vi "Scripting_UpdateViFromTemplate.vi"(0 "ViRef":refnum<vi>, 1 "TemplateVI(Path or Ref)":variant, 5 "error in (no error)":errorcluster) -> (15 "TemplateVersionUsed":string, 19 "error out":errorcluster={"status"=TRUE, "code"=1055, "source"="Property Node in Scripting_ConvertBaseClassToSubClass.vi"})   [LabVIEW 2020]
uses:
  <vilib>/Utility/miscctls.llb/LVRectTypeDef.ctl
  <vilib>/Utility/miscctls.llb/LVPositionTypeDef.ctl
  <vilib>/Utility/traverseref.llb/TRef TravTarget.ctl
  b5d46679-8400-4ee0-8a03-e36cc4015ed4.vi
  Scripting.lvclass
  <vilib>/Utility/traverseref.llb/VI Scripting - Traverse.lvlib
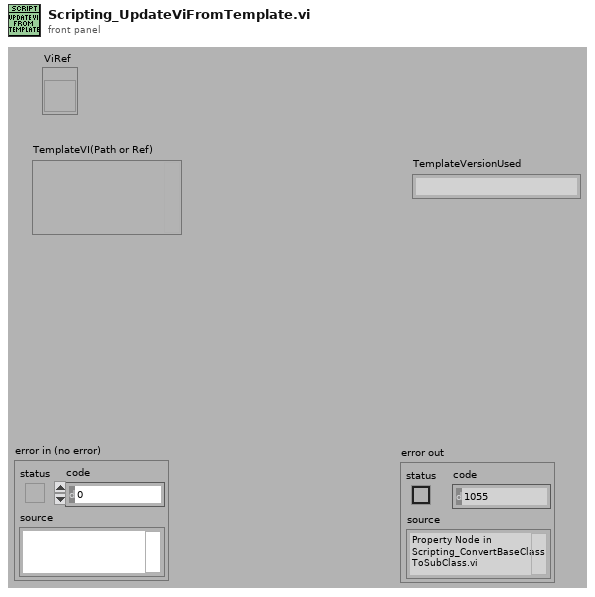
[diagram p1: front panel]
types:
  T1 = typedef "LVRectTypeDef.ctl" = cluster{"Left":i16, "Top":i16, "Right":i16, "Bottom":i16}
  T2 = typedef "LVPositionTypeDef.ctl" = cluster{"Left":i32, "Top":i32}
  T3 = cluster{"ViRef":refnum<vi>, "TemplateRef":refnum<vi>, "ConnectorPaneSettings":cluster{i32, "Wire Rule":enum16{"Invalid Wire Rule", "Required", "Recommended", "Optional", "Dynamic Dispatch"}}[], "ConnectorPaneControlsLabels":string[], "ViClassPath":path, "TemplateViClassPath":path, "ViRootBaseClassPath":path, "TemplateRootBaseClassPath":path, "ClassName":string, "TemplateMemberDataPath":path, "TemplateFile":path, "TemplateVersionUsed":string, "Class":refnum<vi>, "TemplateClassName":string, "permissions":i16, "TemplateClass":refnum<vi>, "Master Bounds Rect":T1, "Visible":bool[], "Controls":refnum<vi>[], "Positions":T2[], "CtrlsNotOnCP":string[]}
  T4 = enum32{"invalid lock state", "Not Locked", "Locked (No Password)", "Password-protected"}
  T5 = typedef "TRef TravTarget.ctl" = enum16{"FP", "BD", "Other"}
  T6 = enum32{"invalid VI type", "Standard VI", "Control VI", "Global VI", "Polymorphic VI", "Configuration VI", "SubSystem", "Facade VI", "Method VI", "Statechart Diagram VI"}
  T7 = enum32{"invalid VI type", "Standard VI", "Control VI", "Global VI", "Polymorphic VI", "Configuration VI", "SubSystem", "Facade VI", "Method VI"}
  T8 = cluster{"Major":u16, "Minor":u16, "Fix":u16, "Build":u16}
  T9 = enum16{"Invalid Wire Rule", "Required", "Recommended", "Optional", "Dynamic Dispatch"}[]
  T10 = cluster{i32, "Wire Rule":enum16{"Invalid Wire Rule", "Required", "Recommended", "Optional", "Dynamic Dispatch"}}
  T11 = cluster{"Position":T2, "Label.Text":string, "Visible":bool, cluster{i32, "Wire Rule":enum16{"Invalid Wire Rule", "Required", "Recommended", "Optional", "Dynamic Dispatch"}}}
  T12 = cluster{"Position":T2, "Label.Text":string, "Visible":bool, cluster{i32, "Wire Rule":enum16{"Invalid Wire Rule", "Required", "Recommended", "Optional", "Dynamic Dispatch"}}}[]
  T13 = cluster{i32, "Wire Rule":enum16{"Invalid Wire Rule", "Required", "Recommended", "Optional", "Dynamic Dispatch"}}[]
  T14 = cluster{"Position":T2, refnum<vi>, "Label.Text":string}
  T15 = cluster{"Position":T2, refnum<vi>, "Label.Text":string}[]
  T16 = enum16{"Invalid Wire Rule", "Required", "Recommended", "Optional", "Dynamic Dispatch"}
  T17 = enum32{"Bad", "Idle", "Run top level", "Running"}
  T18 = typedef "LVPointTypeDef.ctl" = cluster{"Horizontal":i16, "Vertical":i16}
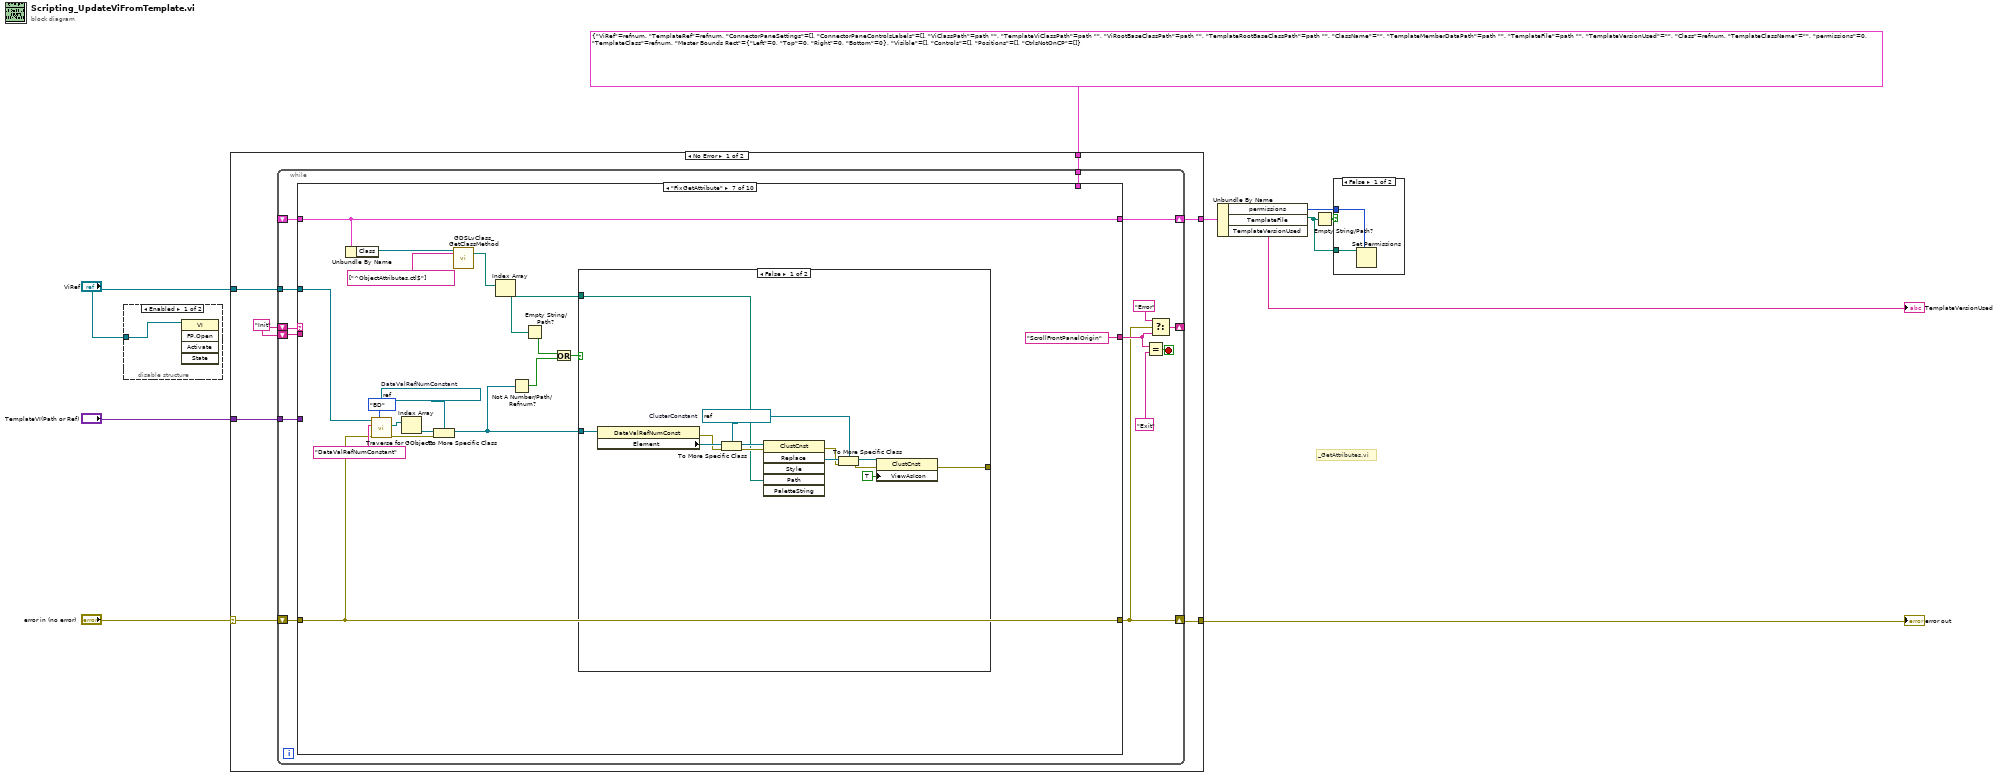
[diagram p0: block diagram]
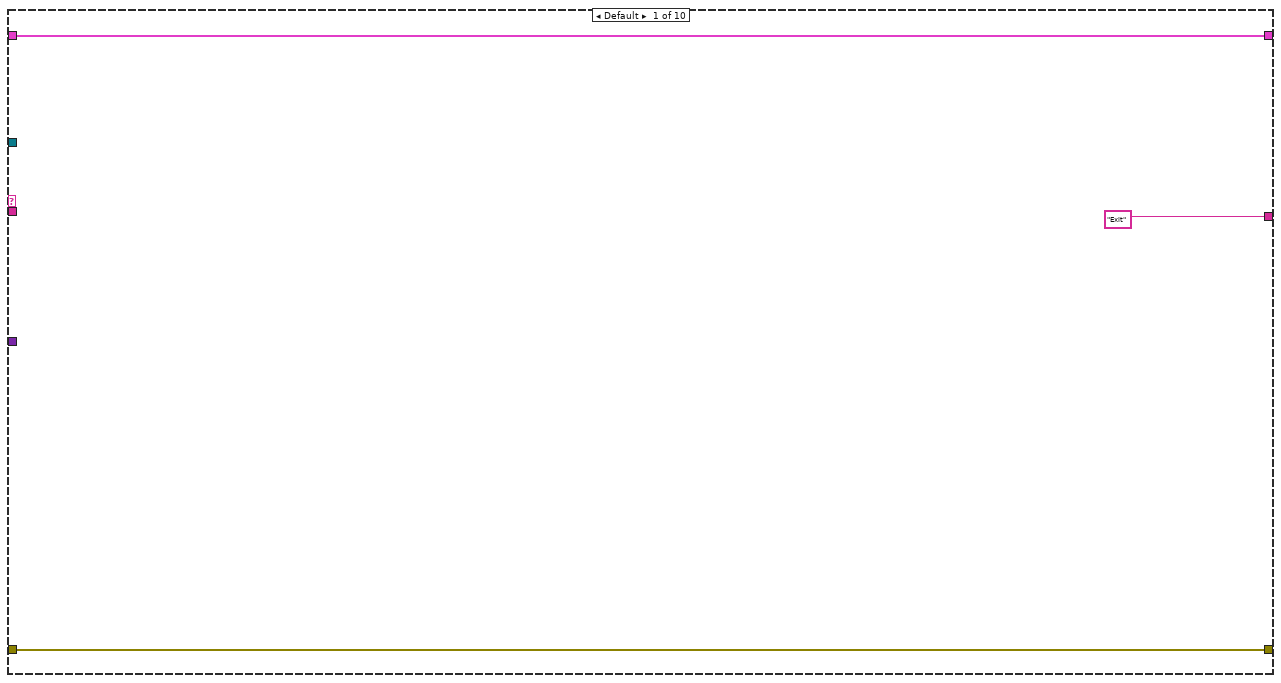
[diagram p4: hidden frame]
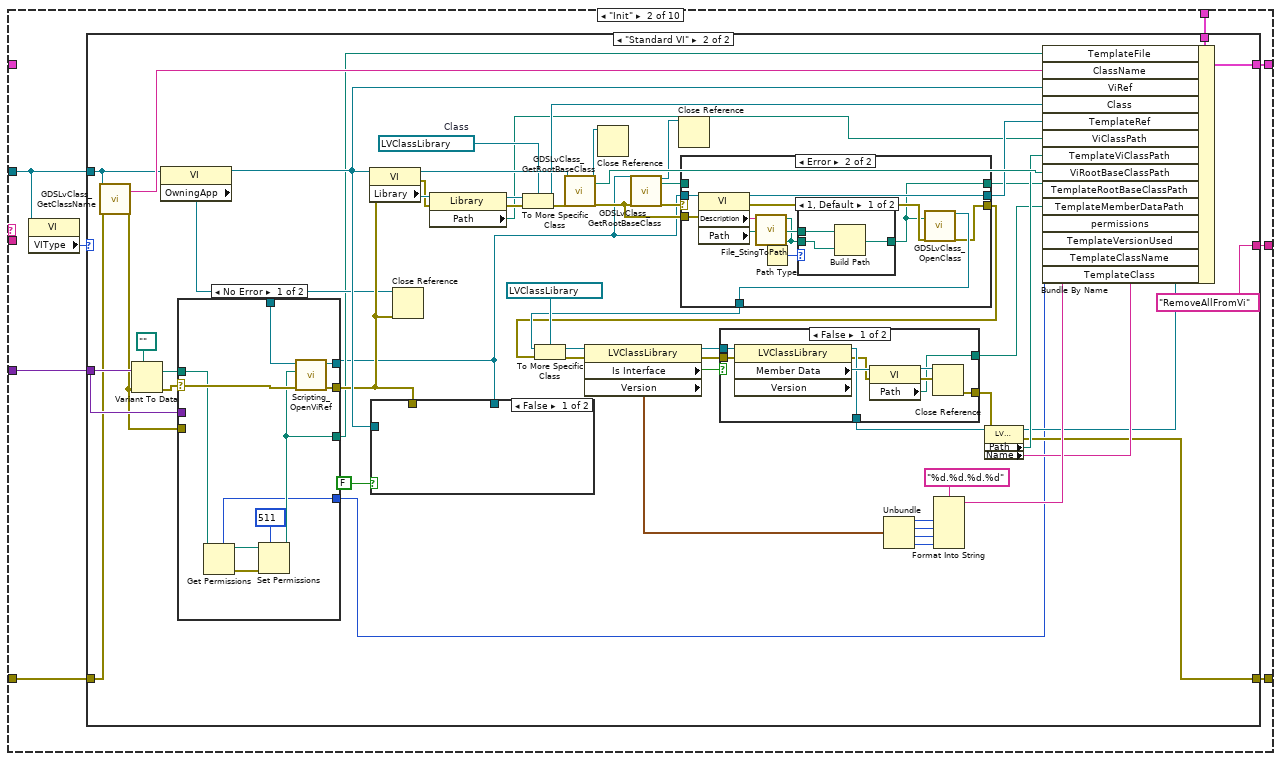
[diagram p5: hidden frame]
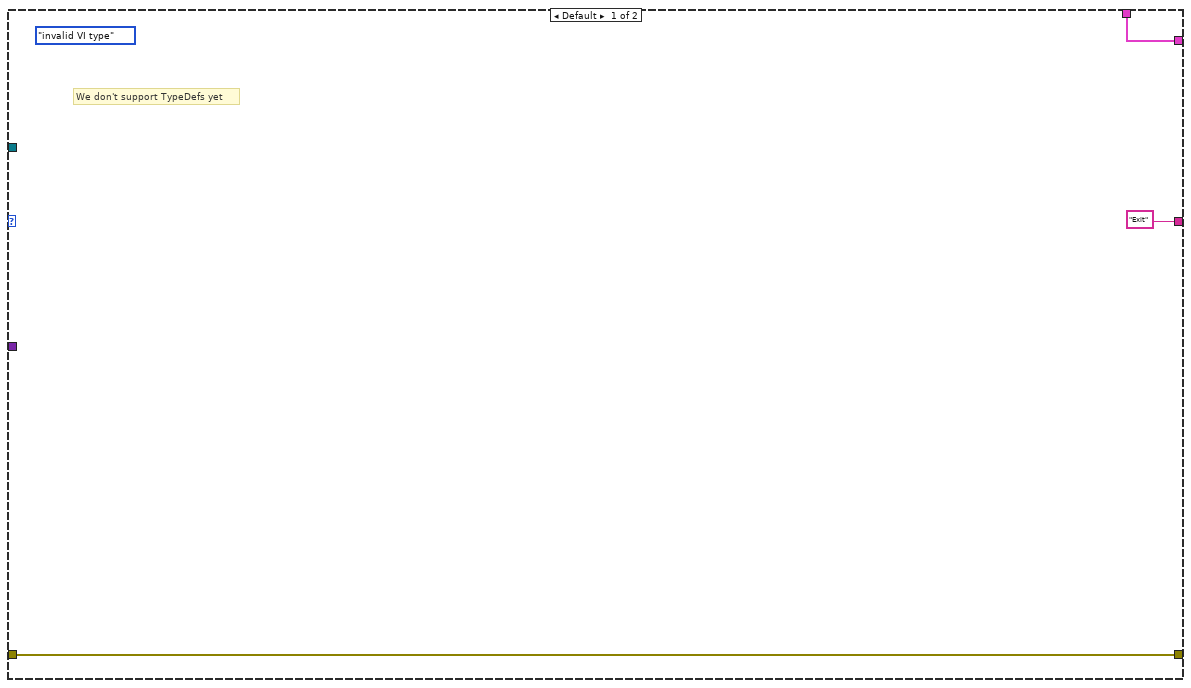
[diagram p6: hidden frame]
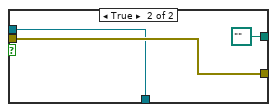
[diagram p7: hidden frame]
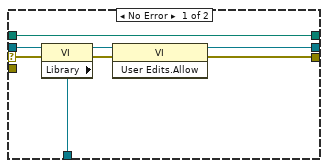
[diagram p8: hidden frame]
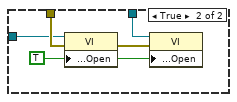
[diagram p10: hidden frame]
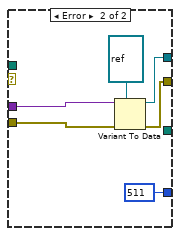
[diagram p11: hidden frame]
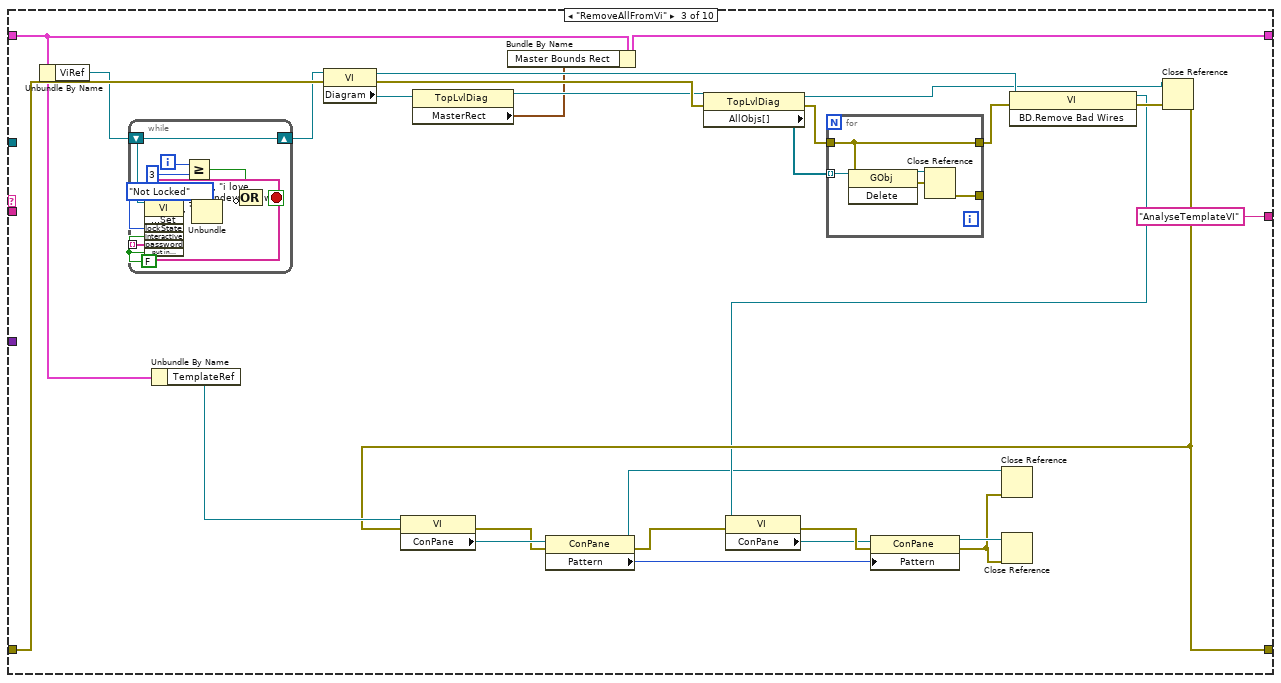
[diagram p12: hidden frame]
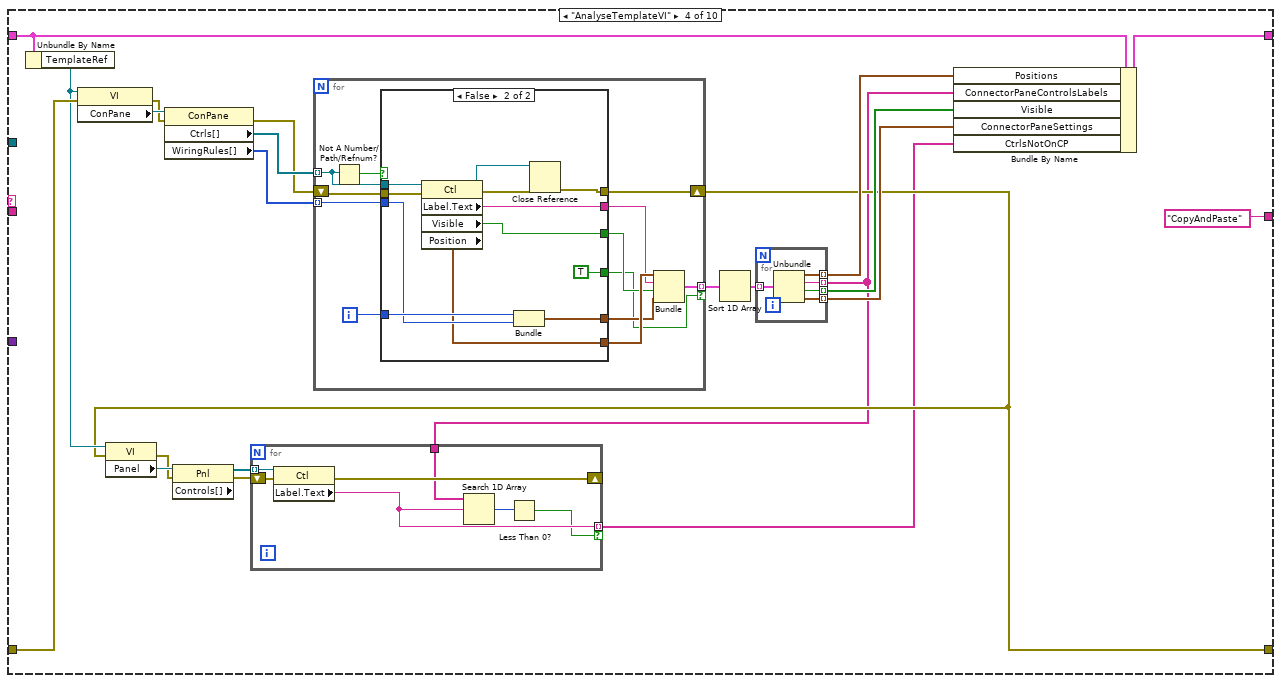
[diagram p13: hidden frame]
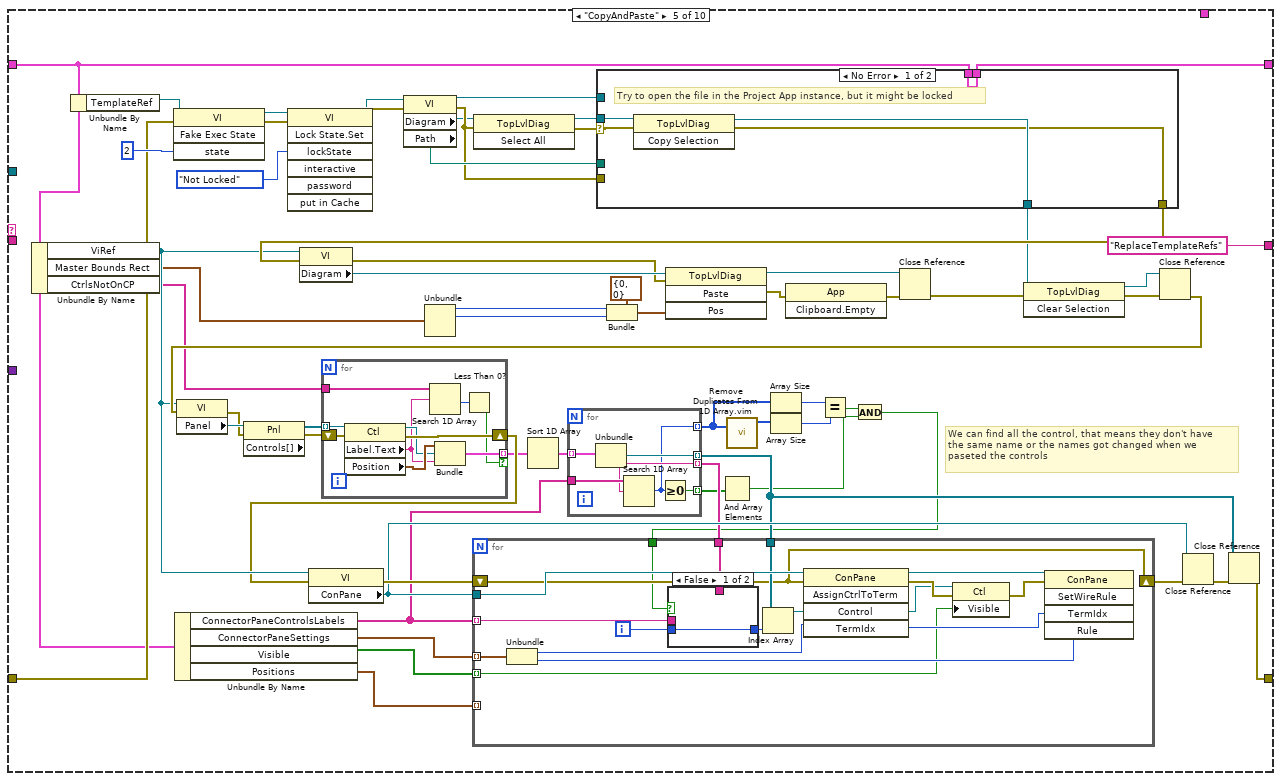
[diagram p15: hidden frame]
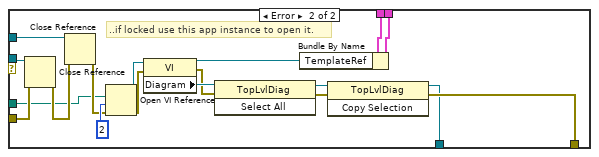
[diagram p16: hidden frame]
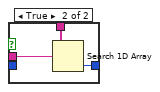
[diagram p17: hidden frame]
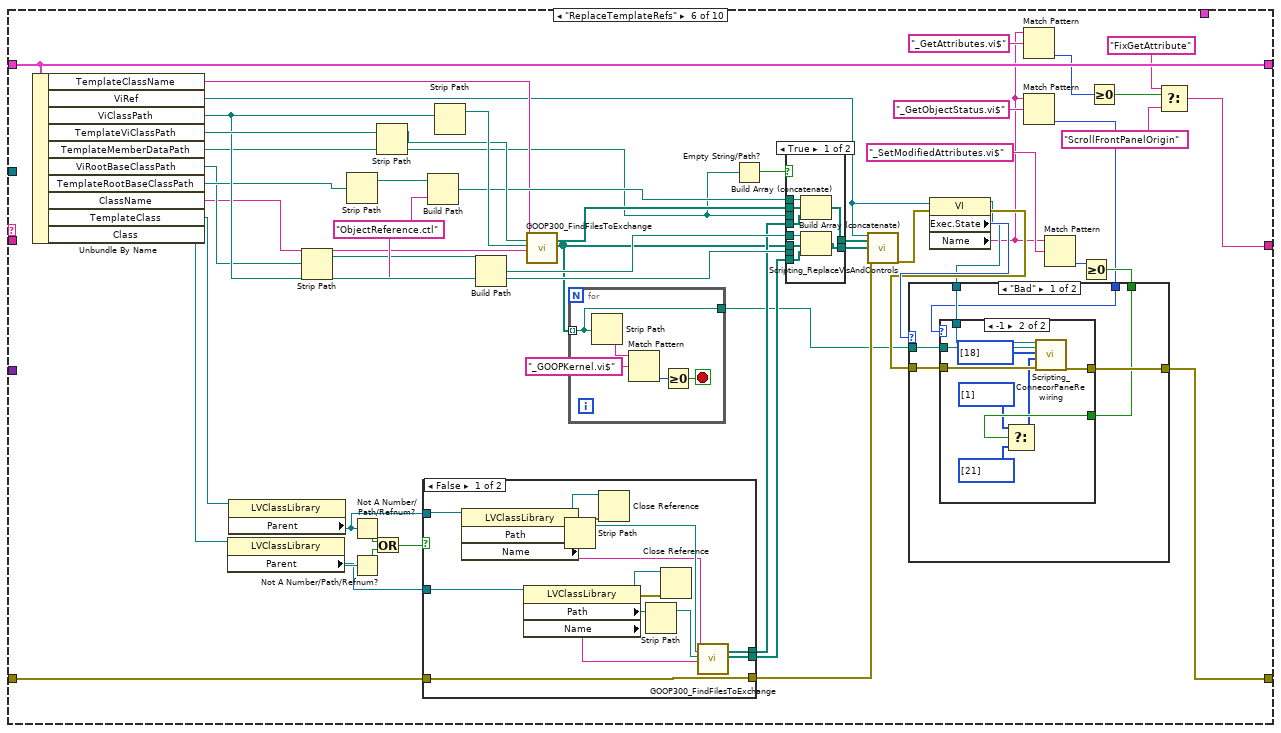
[diagram p18: hidden frame]
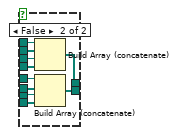
[diagram p19: hidden frame]
diagram:
  # "_GetAttributes.vi"
  n1 = disable-structure shown="Enabled" {
    disable-tunnel: "ViRef" -> [w11 _]
    frame Enabled {
      n2 = invoke class="VI" method="FP.Open"(reference=w11) -> ()  [unwired: 4 in, 5 out]
    }
    frame Disabled {
    }
  }
  n3 = case shown="No Error" "error in (no error)" {
    selector: "error in (no error)" -> [w13 w635]
    tunnel: [w18 w635] -> w10
    tunnel: T3 {"ViRef"=refnum, "TemplateRef"=refnum, "ConnectorPaneSettings"=[], "ConnectorPaneControlsLabels"=[], "ViClassPath"=path "", "TemplateViClassPath"=path "", "ViRootBaseClassPath"=path "", "TemplateRootBaseClassPath"=path "", "ClassName"="", "TemplateMemberDataPath"=path "", "TemplateFile"=path "", "TemplateVersionUsed"="", "Class"=refnum, "TemplateClassName"="", "permissions"=0, "TemplateClass"=refnum, "Master Bounds Rect"={"Left"=0, "Top"=0, "Right"=0, "Bottom"=0}, "Visible"=[], "Controls"=[], "Positions"=[], "CtrlsNotOnCP"=[]} -> [w17 _]
    tunnel: "ViRef" -> [w16 _]
    tunnel: "TemplateVI(Path or Ref)" -> [w15 _]
    tunnel: [w12 _] -> w6
    frame No Error {
      w14 = "Init"
      n4 = while {
        shift-right: [w20] -> w18
        shift-left: w13 -> [w22]
        shift-right: [w32] -> _
        shift-left: w14 -> [w27]
        shift-right: [w21] -> w12
        shift-left: _ -> [w26]
        tunnel: w16 -> [w24]
        tunnel: w17 -> [w25]
        tunnel: w15 -> [w23]
        shift-left: w14 -> [w19]
        stop <- w31 stop-if-true
        n5 = case shown="\"FixGetAttribute\"" w27 {
          tunnel: w22 -> [w35 w39 w186 w221 w310 w394 w500 w559 w590 w596]
          tunnel: [w35 w38 w167 w205 w280 w392 w500 w559 w589 w599] -> w20
          tunnel: ["Exit" w43 "AnalyseTemplateVI" "CopyAndPaste" "ReplaceTemplateRefs" w381 "ScrollFrontPanelOrigin" "SaveVI" "CloseReferences" "Exit"] -> w28
          tunnel: [w33 w42 w173 w222 w302 w393 w498 w528 w592 w595] -> w21
          tunnel: w26 -> [w33 _ w171 w223 w296 w393 w498 w528 w592 w595]
          tunnel: w24 -> [_ w37 _ _ _ _ w501 w521 _ w604]
          tunnel: w25 -> [_ w41 _ _ _ _ _ _ _ _]
          tunnel: w23 -> [_ w40 _ _ _ _ _ _ _ w606]
          tunnel: w19 -> [_ _ _ _ _ _ _ _ _ w594]
          frame Default {
          }
          frame "Init" {
            n6 = property class="VI"(reference=w37) -> ("VIType"=w36:T6)  [unwired: 1 in, 2 out]
            n7 = case shown="\"Standard VI\"" w36 {
              tunnel: ["Exit" "RemoveAllFromVi"] -> w43
              tunnel: [w46 w102] -> w42
              tunnel: w41 -> [w46 w101]
              tunnel: w40 -> [_ w97]
              tunnel: w39 -> [w44 w88]
              tunnel: [w44 w64] -> w38
              tunnel: w37 -> [_ w62]
              frame Default {
                (unwired) T7."invalid VI type" ("VIType")
                # "We don't support TypeDefs yet"
              }
              frame "Standard VI" {
                w68 = refnum<vi> refnum  # Class
                n8 = call "GDSLvClass_GetClassName.vi"("ViRef/Path,LvClassRef/Path"=w62, "error in (no error)"=w88) -> ("ClassName(without .lvclass)"=w87:string, "error out"=w85:errorcluster)  [unwired: 15 in, 1 out]
                n9 = Variant To Data(error in=w85, type=path "", Variant=w97) -> (data=w98:path, error out=w99:errorcluster)
                n10 = property class="VI"(reference=w62) -> (reference out=w82:refnum<vi>, "OwningApp"=w80:refnum<vi>)  [unwired: 1 in, 1 out]
                n11 = case shown="No Error" w99 {
                  selector: w99 -> [w152 _]
                  tunnel: w98 -> [w145 _]
                  tunnel: [w151 w155] -> w53
                  tunnel: [w150 w154] -> w81
                  tunnel: w85 -> [_ w158]
                  tunnel: w97 -> [_ w157]
                  tunnel: w80 -> [w149 _]
                  tunnel: [w147 _] -> w77
                  tunnel: [w143 i16 511 ("permissions")] -> w60
                  frame No Error {
                    n12 = Get Permissions(11:w145) -> (0:w146:errorcluster, 3:w144:path, 5:w143:i16)  [unwired: 1 in, 2 out]
                    n13 = Set Permissions(7:i16 511 ("permissions"), 8:w146, 11:w144) -> (3:w147:path)  [unwired: 2 in, 1 out]
                    n14 = call "Scripting_OpenViRef.vi"("error in"=w152, "ViPath/ViName/Viref"=w147, "AppRef"=w149) -> ("error out"=w150:errorcluster, "vi reference"=w151:refnum<vi>)  [unwired: 6 in, 1 out]
                  }
                  frame Error {
                    n15 = Variant To Data(error in=w158, type=refnum<vi> refnum ("ViRef"), Variant=w157) -> (data=w155:refnum<vi>, error out=w154:errorcluster)
                  }
                }
                n16 = property class="VI"(reference=w82, error in=w81) -> (reference out=w95:refnum<vi>, error out=w84:errorcluster, "Library"=w96:refnum<vi>)
                n17 = case shown="False" FALSE {
                  tunnel: w81 -> [_ w140]
                  tunnel: w53 -> [_ w139]
                  tunnel: w82 -> [_ w138]
                  frame False {
                  }
                  frame True {
                    w141 = TRUE ("Front Panel Window:Open")
                    n18 = property class="VI"(reference=w138, error in=w140, "Front Panel.Open"=w141) -> (error out=w142:errorcluster)  [unwired: 1 out]
                    n19 = property class="VI"(reference=w139, error in=w142, "Front Panel.Open"=w141) -> ()  [unwired: 2 out]
                  }
                }
                n20 = Close Reference(reference=w80, error in (no error)=w81) -> ()  [unwired: 1 out]
                n21 = property class="Library"(reference=w96, error in=w84) -> (reference out=w70:refnum<vi>, error out=w69:errorcluster, "Path"=w59:path)
                n22 = To More Specific Class(target class=w68, reference=w70, error in=w69) -> (specific class reference=w66:refnum<vi>, error out=w67:errorcluster)
                n23 = call "GDSLvClass_GetRootBaseClass.vi"("ViRef/Path,LvClassRef/Path"=w95, "error in (no error)"=w67) -> ("RootBaseClassRef"=w94:refnum<vi>, "RootBaseClassPath"=w93:path, "error out"=w57:errorcluster)  [unwired: 11 in, 4 out]
                n24 = Close Reference(reference=w94) -> ()  [unwired: 1 in, 1 out]
                n25 = call "GDSLvClass_GetRootBaseClass.vi"("ViRef/Path,LvClassRef/Path"=w53, "error in (no error)"=w57) -> ("RootBaseClassRef"=w61:refnum<vi>, "RootBaseClassPath"=w56:path, "error out"=w58:errorcluster)  [unwired: 11 in, 4 out]
                n26 = Close Reference(reference=w61) -> ()  [unwired: 1 in, 1 out]
                n27 = case shown="Error" w58 {
                  selector: w58 -> [w117 _]
                  tunnel: [w123 w129] -> w91
                  tunnel: [w122 w133] -> w79
                  tunnel: [w120 w128] -> w78
                  tunnel: w53 -> [w118 w133]
                  tunnel: w57 -> [_ w132]
                  tunnel: w56 -> [w116 _]
                  tunnel: [w116 w124] -> w55
                  frame No Error {
                    n28 = property class="VI"(reference=w118, error in=w117) -> (reference out=w119:refnum<vi>, error out=w121:errorcluster, "Library"=w123:refnum<vi>)
                    n29 = invoke class="VI" method="User Edits.Allow"(reference=w119, error in=w121) -> (reference out=w122:refnum<vi>, error out=w120:errorcluster)  [unwired: 1 in, 1 out]
                  }
                  frame Error {
                    n30 = property class="VI"(reference=w133, error in=w132) -> (error out=w130:errorcluster, "Description"=w131:string, "Path"=w127:path)  [unwired: 1 out]
                    n31 = call "File_StingToPath.vi"("Description"=w131) -> ("Path"=w126:path)  [unwired: 10 in]
                    n32 = Path Type(1:w126) -> (0:w125:i16)
                    n33 = case shown="1, Default" w125 {
                      tunnel: w126 -> [w134 w137]
                      tunnel: [w136 w137] -> w124
                      tunnel: w127 -> [w135 _]
                      frame 1, Default {
                        n34 = Build Path(base path=w135, name or relative path=w134) -> (appended path=w136:path)
                      }
                      frame 0 {
                      }
                    }
                    n35 = call "GDSLvClass_OpenClass.vi"("ClassToOpen"=w124, "error in (no error)"=w130) -> ("LVClass.Open"=w129:refnum<vi>, "error out"=w128:errorcluster)  [unwired: 16 in]
                  }
                }
                n36 = To More Specific Class(target class=refnum<vi> refnum ("LVClass.Open"), reference=w91, error in=w78) -> (specific class reference=w52:refnum<vi>, error out=w51:errorcluster)
                n37 = property class="LVClassLibrary"(reference=w52, error in=w51) -> (reference out=w50:refnum<vi>, error out=w49:errorcluster, "Is Interface"=w47:bool, "Version"=w48:T8)
                n38 = case shown="False" w47 {
                  tunnel: [w110 w113] -> w90
                  tunnel: [w109 w115] -> w89
                  tunnel: [w106 path "" ("Path")] -> w54
                  tunnel: w50 -> [w105 w113]
                  tunnel: w49 -> [w104 w115]
                  frame False {
                    n39 = property class="LVClassLibrary" props=["Member Data", "Version"](reference=w105, error in=w104) -> (reference out=w110:refnum<vi>, error out=w108:errorcluster, "Member Data"=w111:refnum<vi>)  [unwired: 1 out]
                    n40 = property class="VI"(reference=w111, error in=w108) -> (reference out=w107:refnum<vi>, error out=w112:errorcluster, "Path"=w106:path)
                    n41 = Close Reference(reference=w107, error in (no error)=w112) -> (error out=w109:errorcluster)
                  }
                  frame True {
                  }
                }
                n42 = Unbundle(w48) -> ("Major"=w76:u16, "Minor"=w75:u16, "Fix"=w74:u16, "Build"=w73:u16)
                n43 = Format Into String(format string="%d.%d.%d.%d", w76, w75, w74, w73) -> (resulting string=w71:string)  [unwired: 2 in, 1 out]
                n44 = property class="LVClassLibrary"(reference=w90, error in=w89) -> (reference out=w63:refnum<vi>, error out=w64:errorcluster, "Path"=w86:path, "Name"=w65:string)
                n45 = Bundle By Name(cluster=w101, "TemplateFile"=w77, "ClassName"=w87, "ViRef"=w82, "Class"=w66, "TemplateRef"=w79, "ViClassPath"=w59, "TemplateViClassPath"=w86, "ViRootBaseClassPath"=w93, "TemplateRootBaseClassPath"=w55, "TemplateMemberDataPath"=w54, "permissions"=w60, "TemplateVersionUsed"=w71, "TemplateClassName"=w65, "TemplateClass"=w63) -> (w102:T3)
              }
            }
          }
          frame "RemoveAllFromVi" {
            n46 = Unbundle By Name(w171) -> ("ViRef"=w177:refnum<vi>)
            n47 = while {
              tunnel: string[] ["goop rules", "i love goteborg", "Endevo Knows Goop!", "kiss"] -> [w195] mode=indexing
              shift-right: [w188] -> w176
              shift-left: w177 -> [w188]
              i -> [w192]
              stop <- w193 stop-if-true
              w196 = FALSE ("Interactive")
              n48 = invoke class="VI" method="Lock State.Set"(reference=w188, "lockState"=T4."Not Locked" ("Lock State"), "interactive"=w196, "password"=w195, "put in Cache"=w196) -> (error out=w194:errorcluster)  [unwired: 2 in, 6 out]
              n49 = Greater Or Equal?(x=w192, y=3) -> (x >= y?=w191:bool)
              n50 = Unbundle(w194) -> ("status"=w189:bool)  [unwired: 2 out]
              n51 = Compound Arithmetic op=OR(w191, invert w189) -> (w193:bool)
            }
            n52 = Unbundle By Name(w171) -> ("TemplateRef"=w168:refnum<vi>)
            n53 = property class="VI"(reference=w176, error in=w186) -> (reference out=w184:refnum<vi>, error out=w181:errorcluster, "Diagram"=w175:refnum<vi>)
            n54 = property class="TopLvlDiag"(reference=w175) -> (reference out=w174:refnum<vi>, "MasterRect"=w172:T1)  [unwired: 1 in, 1 out]
            n55 = Bundle By Name(cluster=w171, "Master Bounds Rect"=w172) -> (w173:T3)
            n56 = property class="TopLvlDiag"(reference=w174, error in=w181) -> (reference out=w179:refnum<vi>, error out=w183:errorcluster, "AllObjs[]"=w182:refnum<vi>[])
            n57 = for {
              tunnel: w183 -> [w200]
              tunnel: w182 -> [w201] mode=indexing
              tunnel: [w200] -> w180
              tunnel: [w198] -> _
              n58 = invoke class="GObj" method="Delete"(reference=w201, error in=w200) -> (reference out=w202:refnum<vi>, error out=w199:errorcluster)  [unwired: 1 in, 1 out]
              n59 = Close Reference(reference=w202, error in (no error)=w199) -> (error out=w198:errorcluster)
            }
            n60 = invoke class="VI" method="BD.Remove Bad Wires"(reference=w184, error in=w180) -> (reference out=w163:refnum<vi>, error out=w185:errorcluster)  [unwired: 1 in, 1 out]
            n61 = Close Reference(reference=w179, error in (no error)=w185) -> (error out=w167:errorcluster)
            n62 = property class="VI"(reference=w168, error in=w167) -> (error out=w169:errorcluster, "ConPane"=w170:refnum<vi>)  [unwired: 1 out]
            n63 = property class="ConPane"(reference=w170, error in=w169) -> (reference out=w161:refnum<vi>, error out=w164:errorcluster, "Pattern"=w162:u32)
            n64 = property class="VI"(reference=w163, error in=w164) -> (error out=w166:errorcluster, "ConPane"=w165:refnum<vi>)  [unwired: 1 out]
            n65 = property class="ConPane"(reference=w165, error in=w166, "Pattern"=w162) -> (reference out=w160:refnum<vi>, error out=w159:errorcluster)
            n66 = Close Reference(reference=w161, error in (no error)=w159) -> ()  [unwired: 1 out]
            n67 = Close Reference(reference=w160, error in (no error)=w159) -> ()  [unwired: 1 out]
          }
          frame "AnalyseTemplateVI" {
            n68 = Unbundle By Name(w223) -> ("TemplateRef"=w206:refnum<vi>)
            n69 = property class="VI"(reference=w206, error in=w221) -> (error out=w216:errorcluster, "ConPane"=w220:refnum<vi>)  [unwired: 1 out]
            n70 = property class="ConPane"(reference=w220, error in=w216) -> (error out=w217:errorcluster, "Ctrls[]"=w219:refnum<vi>[], "WiringRules[]"=w218:T9)  [unwired: 1 out]
            n71 = for {
              tunnel: w219 -> [w246] mode=indexing
              tunnel: w218 -> [w244] mode=indexing
              shift-right: [w243] -> w205
              shift-left: w217 -> [w247]
              tunnel: [w238] -> w215 mode=indexing if=w237
              i -> [w245]
              n72 = Not A Number/Path/Refnum?(number/path/refnum=w246) -> (NaN/Path/Refnum?=w248:bool)
              n73 = case shown="False" w248 {
                tunnel: w247 -> [w249 w261]
                tunnel: w246 -> [_ w260]
                tunnel: w245 -> [_ w259]
                tunnel: w244 -> [_ w258]
                tunnel: [w249 w255] -> w243
                tunnel: [_ w254] -> w241
                tunnel: [_ w253] -> w240
                tunnel: [_ w252] -> w239
                tunnel: [_ w251] -> w242
                tunnel: [_ TRUE] -> w237
                frame True {
                }
                frame False {
                  n74 = property class="Ctl"(reference=w260, error in=w261) -> (reference out=w256:refnum<vi>, error out=w257:errorcluster, "Label.Text"=w254:string, "Visible"=w253:bool, "Position"=w251:T2)
                  n75 = Bundle(w259, "Wire Rule"=w258) -> (w252:T10)  [unwired: 1 in]
                  n76 = Close Reference(reference=w256, error in (no error)=w257) -> (error out=w255:errorcluster)
                }
              }
              n77 = Bundle("Position"=w242, "Label.Text"=w241, "Visible"=w240, w239) -> (w238:T11)  [unwired: 1 in]
            }
            n78 = property class="VI"(reference=w206, error in=w205) -> (error out=w209:errorcluster, "Panel"=w210:refnum<vi>)  [unwired: 1 out]
            n79 = property class="Pnl"(reference=w210, error in=w209) -> (error out=w208:errorcluster, "Controls[]"=w207:refnum<vi>[])  [unwired: 1 out]
            n80 = Sort 1D Array(array=w215) -> (sorted array=w214:T12)
            n81 = for {
              tunnel: w214 -> [w236] mode=indexing
              tunnel: [w235] -> w213 mode=indexing
              tunnel: [w234] -> w204 mode=indexing
              tunnel: [w233] -> w212 mode=indexing
              tunnel: [w232] -> w211 mode=indexing
              n82 = Unbundle(w236) -> ("Position"=w235:T2, "Label.Text"=w234:string, "Visible"=w233:bool, w232:T10)
            }
            n83 = for {
              tunnel: w207 -> [w229] mode=indexing
              shift-right: [w230] -> _
              shift-left: w208 -> [w231]
              tunnel: w204 -> [w228]
              tunnel: [w226] -> w203 mode=indexing if=w225
              n84 = property class="Ctl"(reference=w229, error in=w231) -> (error out=w230:errorcluster, "Label.Text"=w226:string)  [unwired: 1 out]
              n85 = Search 1D Array(1D array=w228, element=w226) -> (index of element=w227:i32)  [unwired: 1 in]
              n86 = Less Than 0?(x=w227) -> (x < 0?=w225:bool)
            }
            n87 = Bundle By Name(cluster=w223, "Positions"=w213, "ConnectorPaneControlsLabels"=w204, "Visible"=w212, "ConnectorPaneSettings"=w211, "CtrlsNotOnCP"=w203) -> (w222:T3)
          }
          frame "CopyAndPaste" {
            # "We can find all the control, that means they don't have\nthe same name or the names got changed when we\npaseted the controls"
            n88 = Unbundle By Name(w296) -> ("ViRef"=w294:refnum<vi>, "Master Bounds Rect"=w288:T1, "CtrlsNotOnCP"=w262:string[])
            n89 = Unbundle By Name(w296) -> ("TemplateRef"=w311:refnum<vi>)
            n90 = invoke class="VI" method="Fake Exec State"(reference=w311, error in=w310, "state"=2 ("State")) -> (reference out=w306:refnum<vi>, error out=w309:errorcluster)  [unwired: 1 in, 2 out]
            n91 = Unbundle By Name(w296) -> ("ConnectorPaneControlsLabels"=w271:string[], "ConnectorPaneSettings"=w315:T13, "Visible"=w279:bool[], "Positions"=w278:T2[])
            n92 = invoke class="VI" method="Lock State.Set"(reference=w306, "lockState"=T4."Not Locked" ("Lock State")) -> (reference out=w307:refnum<vi>)  [unwired: 5 in, 6 out]
            n93 = property class="VI"(reference=w307, error in=w309) -> (reference out=w295:refnum<vi>, error out=w303:errorcluster, "Diagram"=w293:refnum<vi>, "Path"=w304:path)
            n94 = Unbundle(w288) -> ("Left"=w287:i16, "Top"=w286:i16)  [unwired: 2 out]
            n95 = invoke class="TopLvlDiag" method="Select All"(reference=w293, error in=w303) -> (reference out=w320:refnum<vi>, error out=w305:errorcluster)  [unwired: 1 in, 1 out]
            n96 = case shown="No Error" w305 {
              selector: w305 -> [w331 _]
              tunnel: w320 -> [w332 w344]
              tunnel: [w328 w339] -> w297
              tunnel: w304 -> [_ w335]
              tunnel: w303 -> [_ w343]
              tunnel: w296 -> [w330 w348]
              tunnel: [w330 w347] -> w302
              tunnel: [w329 w338] -> w284
              tunnel: w295 -> [_ w345]
              frame No Error {
                # "Try to open the file in the Project App instance, but it might be locked"
                n97 = invoke class="TopLvlDiag" method="Copy Selection"(reference=w332, error in=w331) -> (reference out=w329:refnum<vi>, error out=w328:errorcluster)  [unwired: 1 in, 1 out]
              }
              frame Error {
                # "..if locked use this app instance to open it."
                n98 = Close Reference(reference=w344, error in (no error)=w343) -> (error out=w342:errorcluster)
                n99 = Close Reference(reference=w345, error in (no error)=w342) -> (error out=w336:errorcluster)
                n100 = Open VI Reference(vi path=w335, options=2, error in (no error)=w336) -> (vi reference=w333:refnum<vi>, error out=w334:errorcluster)  [unwired: 3 in]
                n101 = property class="VI"(reference=w333, error in=w334) -> (reference out=w346:refnum<vi>, error out=w349:errorcluster, "Diagram"=w350:refnum<vi>)
                n102 = invoke class="TopLvlDiag" method="Select All"(reference=w350, error in=w349) -> (reference out=w341:refnum<vi>, error out=w340:errorcluster)  [unwired: 1 in, 1 out]
                n103 = Bundle By Name(cluster=w348, "TemplateRef"=w346) -> (w347:T3)
                n104 = invoke class="TopLvlDiag" method="Copy Selection"(reference=w341, error in=w340) -> (reference out=w338:refnum<vi>, error out=w339:errorcluster)  [unwired: 1 in, 1 out]
              }
            }
            n105 = property class="VI"(reference=w294, error in=w297) -> (error out=w289:errorcluster, "Diagram"=w290:refnum<vi>)  [unwired: 1 out]
            n106 = Bundle(cluster=T2 {"Left"=0, "Top"=0} ("Position"), "Left"=w287, "Top"=w286) -> (w291:T2)
            n107 = invoke class="TopLvlDiag" method="Paste"(reference=w290, error in=w289, "Pos"=w291) -> (reference out=w300:refnum<vi>, error out=w299:errorcluster)  [unwired: 1 in, 2 out]
            n108 = invoke class="App" method="Clipboard.Empty"(error in=w299) -> (error out=w301:errorcluster)  [unwired: 2 in, 2 out]
            n109 = Close Reference(reference=w300, error in (no error)=w301) -> (error out=w283:errorcluster)
            n110 = invoke class="TopLvlDiag" method="Clear Selection"(reference=w284, error in=w283) -> (reference out=w285:refnum<vi>, error out=w282:errorcluster)  [unwired: 1 in, 1 out]
            n111 = Close Reference(reference=w285, error in (no error)=w282) -> (error out=w298:errorcluster)
            n112 = property class="VI"(reference=w294, error in=w298) -> (error out=w317:errorcluster, "Panel"=w318:refnum<vi>)  [unwired: 1 out]
            n113 = property class="Pnl"(reference=w318, error in=w317) -> (error out=w316:errorcluster, "Controls[]"=w274:refnum<vi>[])  [unwired: 1 out]
            n114 = for {
              tunnel: w274 -> [w358] mode=indexing
              shift-right: [w359] -> w277
              shift-left: w316 -> [w360]
              tunnel: [w355] -> w276 mode=indexing if=w351
              tunnel: w262 -> [w354]
              n115 = property class="Ctl"(reference=w358, error in=w360) -> (reference out=w356:refnum<vi>, error out=w359:errorcluster, "Label.Text"=w353:string, "Position"=w357:T2)
              n116 = Search 1D Array(1D array=w354, element=w353) -> (index of element=w352:i32)  [unwired: 1 in]
              n117 = Bundle("Position"=w357, w356, "Label.Text"=w353) -> (w355:T14)  [unwired: 1 in]
              n118 = Less Than 0?(x=w352) -> (x < 0?=w351:bool)
            }
            n119 = property class="VI"(reference=w294, error in=w277) -> (error out=w319:errorcluster, "ConPane"=w313:refnum<vi>)  [unwired: 1 out]
            n120 = Sort 1D Array(array=w276) -> (sorted array=w275:T15)
            n121 = for {
              tunnel: w275 -> [w327] mode=indexing
              tunnel: [w326] -> w273 mode=indexing
              tunnel: [w324] -> w272 mode=indexing
              tunnel: w271 -> [w325]
              tunnel: [w323] -> w270 mode=indexing
              tunnel: [w322] -> w268 mode=indexing
              n122 = Unbundle(w327) -> (w326:refnum<vi>, "Label.Text"=w324:string)  [unwired: 1 out]
              n123 = Search 1D Array(1D array=w325, element=w324) -> (index of element=w322:i32)  [unwired: 1 in]
              n124 = Greater Or Equal To 0?(x=w322) -> (x >= 0?=w323:bool)
            }
            n125 = And Array Elements(Boolean array=w270) -> (logical AND=w264:bool)
            n126 = call "Remove Duplicates From 1D Array.vim"("array"=w268) -> ("array with duplicates removed"=w269:i32[])  [unwired: 10 in]
            n127 = Array Size(array=w268) -> (size(s)=w267:i32)
            n128 = Array Size(array=w269) -> (size(s)=w266:i32)
            n129 = Equal?(x=w267, y=w266) -> (x = y?=w265:bool)
            n130 = And(x=w265, y=w264) -> (x .and. y?=w263:bool)
            n131 = for {
              shift-right: [w363] -> w314
              shift-left: w319 -> [w363]
              tunnel: w313 -> [w375]
              tunnel: w271 -> [w374] mode=indexing
              tunnel: w272 -> [w373]
              tunnel: w273 -> [w372]
              tunnel: w315 -> [w370] mode=indexing
              tunnel: w279 -> [w364] mode=indexing
              tunnel: w278 -> [_] mode=indexing
              tunnel: w263 -> [w362]
              i -> [w361]
              n132 = Unbundle(w370) -> (w369:i32, "Wire Rule"=w368:T16)
              n133 = case shown="False" w362 {
                tunnel: [w377 w380] -> w376
                tunnel: w374 -> [_ w379]
                tunnel: w373 -> [_ w378]
                tunnel: w361 -> [w377 _]
                frame False {
                }
                frame True {
                  n134 = Search 1D Array(1D array=w378, element=w379) -> (index of element=w380:i32)  [unwired: 1 in]
                }
              }
              n135 = Index Array(array=w372, index=w376) -> (element=w365:refnum<vi>)
              n136 = invoke class="ConPane" method="AssignCtrlToTerm"(reference=w375, error in=w363, "Control"=w365, "TermIdx"=w369) -> (reference out=w371:refnum<vi>, error out=w366:errorcluster)  [unwired: 1 in, 3 out]
              n137 = property class="Ctl"(reference=w365, error in=w366, "Visible"=w364) -> (error out=w367:errorcluster)  [unwired: 1 out]
              n138 = invoke class="ConPane" method="SetWireRule"(reference=w371, error in=w367, "TermIdx"=w369, "Rule"=w368) -> ()  [unwired: 1 in, 5 out]
            }
            n139 = Close Reference(reference=w313, error in (no error)=w314) -> (error out=w281:errorcluster)
            n140 = Close Reference(reference=w273, error in (no error)=w281) -> (error out=w280:errorcluster)
          }
          frame "ReplaceTemplateRefs" {
            w422 = "ObjectReference.ctl" ("name or relative path")
            n141 = Unbundle By Name(w393) -> ("TemplateClassName"=w417:string, "ViRef"=w404:refnum<vi>, "ViClassPath"=w425:path, "TemplateViClassPath"=w426:path, "TemplateMemberDataPath"=w389:path, "ViRootBaseClassPath"=w419:path, "TemplateRootBaseClassPath"=w424:path, "ClassName"=w416:string, "TemplateClass"=w406:refnum<vi>, "Class"=w405:refnum<vi>)
            n142 = property class="LVClassLibrary"(reference=w405) -> (reference out=w415:refnum<vi>, "Parent"=w410:refnum<vi>)  [unwired: 1 in, 1 out]
            n143 = property class="LVClassLibrary"(reference=w406) -> ("Parent"=w411:refnum<vi>)  [unwired: 1 in, 2 out]
            n144 = Strip Path(path=w419) -> (stripped path=w418:path)  [unwired: 1 out]
            n145 = Strip Path(path=w424) -> (stripped path=w423:path)  [unwired: 1 out]
            n146 = Not A Number/Path/Refnum?(number/path/refnum=w411) -> (NaN/Path/Refnum?=w414:bool)
            n147 = Not A Number/Path/Refnum?(number/path/refnum=w415) -> (NaN/Path/Refnum?=w413:bool)
            n148 = Or(x=w414, y=w413) -> (x .or. y?=w412:bool)
            n149 = Strip Path(path=w426) -> (stripped path=w427:path)  [unwired: 1 out]
            n150 = case shown="False" w412 {
              tunnel: w411 -> [w474 w489]
              tunnel: w410 -> [w486 w488]
              tunnel: [w480 _] -> w409
              tunnel: [w479 _] -> w408
              tunnel: w394 -> [w478 w487]
              tunnel: [w478 w487] -> w407
              frame False {
                n151 = property class="LVClassLibrary"(reference=w474) -> (reference out=w476:refnum<vi>, error out=w475:errorcluster, "Path"=w477:path, "Name"=w472:string)  [unwired: 1 in]
                n152 = property class="LVClassLibrary"(reference=w486) -> (reference out=w484:refnum<vi>, error out=w485:errorcluster, "Path"=w483:path, "Name"=w481:string)  [unwired: 1 in]
                n153 = Strip Path(path=w477) -> (stripped path=w473:path)  [unwired: 1 out]
                n154 = Close Reference(reference=w476, error in (no error)=w475) -> ()  [unwired: 1 out]
                n155 = Strip Path(path=w483) -> (stripped path=w482:path)  [unwired: 1 out]
                n156 = Close Reference(reference=w484, error in (no error)=w485) -> ()  [unwired: 1 out]
                n157 = call "GOOP300_FindFilesToExchange.vi"("OldClassName(Prefix or suffix for some VIs)"=w472, "OldFolderPath"=w473, "NewFolderPath"=w482, "NewClassName(Prefix or suffix for some VIs)"=w481) -> ("OldFiles"=w480:path[], "NewFileArray"=w479:path[])  [unwired: 2 in, 12 out]
              }
              frame True {
                n158 = Close Reference(reference=w488) -> ()  [unwired: 1 in, 1 out]
                n159 = Close Reference(reference=w489) -> ()  [unwired: 1 in, 1 out]
              }
            }
            n160 = Build Path(base path=w423, name or relative path=w422) -> (appended path=w421:path)
            n161 = Strip Path(path=w425) -> (stripped path=w428:path)  [unwired: 1 out]
            n162 = Build Path(base path=w418, name or relative path=w422) -> (appended path=w420:path)
            n163 = call "GOOP300_FindFilesToExchange.vi"("OldClassName(Prefix or suffix for some VIs)"=w417, "OldFolderPath"=w427, "NewFolderPath"=w428, "NewClassName(Prefix or suffix for some VIs)"=w416) -> ("OldFiles"=w431:path[], "NewFileArray"=w400:path[])  [unwired: 2 in, 12 out]
            n164 = for {
              tunnel: w400 -> [w450] mode=indexing
              tunnel: [w450] -> w399
              stop <- w451 stop-if-true
              n165 = Strip Path(path=w450) -> (name=w454:string)  [unwired: 1 out]
              n166 = Match Pattern(string=w454, regular expression="_GOOPKernel.vi$") -> (offset past match=w452:i32)  [unwired: 1 in, 3 out]
              n167 = Greater Or Equal To 0?(x=w452) -> (x >= 0?=w451:bool)
            }
            n168 = Empty String/Path?(string/path=w389) -> (empty?=w388:bool)
            n169 = case shown="True" w388 {
              tunnel: w431 -> [w439 w449]
              tunnel: [w438 w448] -> w430
              tunnel: [w437 w447] -> w429
              tunnel: w425 -> [_ w446]
              tunnel: w421 -> [w436 w445]
              tunnel: w420 -> [w435 w444]
              tunnel: w409 -> [w434 w443]
              tunnel: w408 -> [w433 w442]
              tunnel: w400 -> [w432 w441]
              tunnel: w389 -> [_ w440]
              frame True {
                n170 = Build Array (concatenate)(w436, w439, w434) -> (w438:path[])
                n171 = Build Array (concatenate)(w435, w432, w433) -> (w437:path[])
              }
              frame False {
                n172 = Build Array (concatenate)(w445, w449, w440, w443) -> (w448:path[])
                n173 = Build Array (concatenate)(w444, w441, w446, w442) -> (w447:path[])
              }
            }
            n174 = call "Scripting_ReplaceVisAndControls.vi"("ViRef"=w404, "OldVIsAndControls"=w430, "NewVIsAndControls"=w429, "error in (no error)"=w407) -> ("error out"=w403:errorcluster)  [unwired: 15 out]
            n175 = property class="VI"(reference=w404, error in=w403) -> (reference out=w398:refnum<vi>, error out=w401:errorcluster, "Exec.State"=w402:T17, "Name"=w386:string)
            n176 = Match Pattern(string=w386, regular expression="_GetAttributes.vi$") -> (offset past match=w385:i32)  [unwired: 1 in, 3 out]
            n177 = Match Pattern(string=w386, regular expression="_GetObjectStatus.vi$") -> (offset past match=w390:i32)  [unwired: 1 in, 3 out]
            n178 = Match Pattern(string=w386, regular expression="_SetModifiedAttributes.vi$") -> (offset past match=w396:i32)  [unwired: 1 in, 3 out]
            n179 = Greater Or Equal To 0?(x=w396) -> (x >= 0?=w395:bool)
            n180 = case shown="\"Bad\"" w402 {
              tunnel: w401 -> [w460 w471]
              tunnel: w399 -> [w459 _]
              tunnel: w398 -> [w458 _]
              tunnel: [w457 w471] -> w392
              tunnel: w395 -> [w456 _]
              tunnel: w390 -> [w455 _]
              frame "Bad" {
                n181 = case shown="-1" w455 {
                  tunnel: w460 -> [w461 w470]
                  tunnel: w459 -> [_ w469]
                  tunnel: w458 -> [_ w468]
                  tunnel: [w461 w466] -> w457
                  tunnel: w456 -> [_ w465]
                  frame 0, Default {
                  }
                  frame -1 {
                    n182 = Select(t=u32[] [1] ("OldConnectorPaneIndex"), s=w465, f=u32[] [21] ("OldConnectorPaneIndex")) -> (s? t:f=w463:u32[])
                    n183 = call "Scripting_ConnecorPaneRewiring.vi"("ViRef"=w468, "SubViThatHasChangedConnectorPane"=w469, "OldConnectorPaneIndex"=u32[] [18], "NewConnectorPaneIndex"=w463, "error in (no error)"=w470) -> ("error out"=w466:errorcluster)  [unwired: 14 in]
                  }
                }
              }
              frame "Idle", Default {
              }
            }
            n184 = Greater Or Equal To 0?(x=w385) -> (x >= 0?=w384:bool)
            n185 = Select(t="FixGetAttribute", s=w384, f="ScrollFrontPanelOrigin") -> (s? t:f=w381:string)
          }
          frame "FixGetAttribute" {
            w499 = refnum<vi> refnum  # DataValRefNumConstant
            n186 = Unbundle By Name(w498) -> ("Class"=w497:refnum<vi>)
            n187 = call <vilib>:"Traverse for GObjects.vi"("Traverse Target"=TRef_TravTarget."BD", "error in (no error)"=w500, "Class Name"="DataValRefNumConstant", "VI Refnum"=w501) -> ("error out"=w506:errorcluster, "References"=w504:refnum<vi>[])  [unwired: 4 in, 2 out]
            n188 = Index Array(array=w504) -> (element=w505:refnum<vi>)  [unwired: 1 in]
            n189 = To More Specific Class(target class=w499, reference=w505, error in=w506) -> (specific class reference=w491:refnum<vi>)  [unwired: 1 out]
            n190 = call "GDSLvClass_GetClassMethod.vi"("Class Refnum In"=w497, "VINames"=string[] ["^ObjectAttributes.ctl$"] ("regular expression")) -> ("ViPaths"=w495:path[])  [unwired: 14 in, 3 out]
            n191 = Index Array(array=w495) -> (element=w490:path)  [unwired: 1 in]
            n192 = Not A Number/Path/Refnum?(number/path/refnum=w491) -> (NaN/Path/Refnum?=w493:bool)
            n193 = Empty String/Path?(string/path=w490) -> (empty?=w494:bool)
            n194 = Or(x=w494, y=w493) -> (x .or. y?=w492:bool)
            n195 = case shown="False" w492 {
              tunnel: w491 -> [w520 _]
              tunnel: w490 -> [w515 _]
              tunnel: [w508 _] -> _
              frame False {
                w511 = refnum<vi> refnum  # ClusterConstant
                n196 = property class="DataValRefNumConst"(reference=w520) -> (error out=w516:errorcluster, "Element"=w519:refnum<vi>)  [unwired: 1 in, 1 out]
                n197 = To More Specific Class(target class=w511, reference=w519, error in=w516) -> (specific class reference=w518:refnum<vi>, error out=w517:errorcluster)
                n198 = invoke class="ClustCnst" method="Replace"(reference=w518, error in=w517, "Path"=w515) -> (error out=w510:errorcluster, "Replace"=w512:refnum<vi>)  [unwired: 3 in, 4 out]
                n199 = To More Specific Class(target class=w511, reference=w512, error in=w510) -> (specific class reference=w513:refnum<vi>, error out=w509:errorcluster)
                n200 = property class="ClustCnst"(reference=w513, error in=w509, "ViewAsIcon"=TRUE ("View As Icon")) -> (error out=w508:errorcluster)  [unwired: 1 out]
              }
              frame True {
              }
            }
          }
          frame "ScrollFrontPanelOrigin" {
            w548 = 100000
            w556 = 100000
            n201 = Unbundle By Name(w528) -> ("TemplateRef"=w527:refnum<vi>)
            n202 = call "Scripting_AlignToConenctorPane.vi"("ViRef In"=w521) -> ("VIRefOut"=w522:refnum<vi>)  [unwired: 9 in, 1 out]
            n203 = property class="VI"(reference=w522) -> ("Panel"=w546:refnum<vi>)  [unwired: 1 in, 2 out]
            n204 = property class="VI"(reference=w527) -> ("Panel"=w558:refnum<vi>)  [unwired: 1 in, 2 out]
            n205 = property class="Pnl"(reference=w558) -> (reference out=w529:refnum<vi>, "Panes[]"=w537:refnum<vi>[])  [unwired: 1 in, 1 out]
            n206 = property class="Pnl"(reference=w546) -> (reference out=w531:refnum<vi>, "Panes[]"=w532:refnum<vi>[])  [unwired: 1 in, 1 out]
            n207 = Index Array(array=w537) -> (element=w557:refnum<vi>)  [unwired: 1 in]
            n208 = Index Array(array=w532) -> (element=w547:refnum<vi>)  [unwired: 1 in]
            n209 = property class="Pane"(reference=w557) -> ("Origin"=w555:T18, "Controls[]"=w539:refnum<vi>[])  [unwired: 1 in, 2 out]
            n210 = property class="Pane"(reference=w547) -> (reference out=w545:refnum<vi>, "Controls[]"=w533:refnum<vi>[])  [unwired: 1 in, 1 out]
            n211 = for {
              tunnel: w539 -> [w584] mode=indexing
              shift-right: [w580] -> w554
              shift-left: w556 -> [w581]
              shift-right: [w578] -> w552
              shift-left: w556 -> [w579]
              shift-right: [w576] -> w523
              shift-left: string[] [] -> [w575]
              n212 = property class="Ctl"(reference=w584) -> ("Left"=w583:i32, "Top"=w582:i32, "Visible"=w577:bool, "Label.Text"=w574:string)  [unwired: 1 in, 2 out]
              n213 = case shown="True" w577 {
                tunnel: [w587 w588] -> w576
                tunnel: w575 -> [w586 w588]
                tunnel: w574 -> [w585 _]
                frame False {
                  n214 = Build Array (concatenate)(w586, w585) -> (w587:string[])
                }
                frame True {
                }
              }
              n215 = Max & Min(x=w583, y=w581) -> (min(x,y)=w580:i32)  [unwired: 1 out]
              n216 = Max & Min(x=w582, y=w579) -> (min(x,y)=w578:i32)  [unwired: 1 out]
            }
            n217 = for {
              tunnel: w533 -> [w571] mode=indexing
              shift-right: [w567] -> w549
              shift-left: w548 -> [w568]
              shift-right: [w565] -> w550
              shift-left: w548 -> [w566]
              tunnel: w523 -> [w563]
              n218 = property class="Ctl"(reference=w571) -> (reference out=w561:refnum<vi>, "Left"=w570:i32, "Top"=w569:i32, "Label.Text"=w564:string)  [unwired: 1 in, 1 out]
              n219 = Search 1D Array(1D array=w563, element=w564) -> (index of element=w562:i32)  [unwired: 1 in]
              n220 = case shown="0, Default" w562 {
                tunnel: w561 -> [w573 _]
                frame 0, Default {
                  n221 = property class="Ctl"(reference=w573, "Visible"=FALSE) -> ()  [unwired: 1 in, 2 out]
                }
                frame -1 {
                }
              }
              n222 = Max & Min(x=w570, y=w568) -> (min(x,y)=w567:i32)  [unwired: 1 out]
              n223 = Max & Min(x=w569, y=w566) -> (min(x,y)=w565:i32)  [unwired: 1 out]
            }
            n224 = Unbundle By Name(w555) -> ("Horizontal"=w553:i16, "Vertical"=w551:i16)
            n225 = Subtract(x=w554, y=w553) -> (x-y=w544:i32)
            n226 = Subtract(x=w552, y=w551) -> (x-y=w543:i32)
            n227 = Subtract(x=w549, y=w544) -> (x-y=w542:i32)
            n228 = Subtract(x=w550, y=w543) -> (x-y=w541:i32)
            n229 = Bundle(w542, w541) -> (w540:cluster{i32, i32})  [unwired: 1 in]
            n230 = property class="Pane"(reference=w545, "Origin"=w540) -> (error out=w534:errorcluster)  [unwired: 1 in, 1 out]
            n231 = Close Reference(reference=w539, error in (no error)=w534) -> (error out=w538:errorcluster)
            n232 = Close Reference(reference=w533, error in (no error)=w534) -> (error out=w535:errorcluster)
            n233 = Close Reference(reference=w537, error in (no error)=w538) -> (error out=w530:errorcluster)
            n234 = Close Reference(reference=w532, error in (no error)=w535) -> (error out=w536:errorcluster)
            n235 = Close Reference(reference=w529, error in (no error)=w530) -> (error out=w525:errorcluster)
            n236 = Close Reference(reference=w531, error in (no error)=w536) -> (error out=w526:errorcluster)
            n237 = stacked-sequence {
              tunnel: w526 -> [_]
              tunnel: w525 -> [_]
              frame #0 {
              }
            }
          }
          frame "SaveVI" {
            n238 = Unbundle By Name(w592) -> ("ViRef"=w591:refnum<vi>)
            n239 = call "Scripting_SaveVi.vi"("error in (no error)"=w590, "VIRefToSaveIn"=w591) -> ("error out"=w589:errorcluster)  [unwired: 8 in, 1 out]
          }
          frame "CloseReferences", "Error" {
            n240 = call "GDSError_LogErrorInformation.vi"("State"=w594, "LocalVariableData"=w595, "error in (no error)"=w596) -> ()  [unwired: 16 in, 1 out]
            n241 = property class="VI"(reference=w604) -> ("Name"=w603:string)  [unwired: 1 in, 2 out]
            n242 = Variant To Data(type=path "", Variant=w606) -> (data=w602:path, error out=w605:errorcluster)  [unwired: 1 in]
            n243 = Strip Path(path=w602) -> (name=w601:string)  [unwired: 1 out]
            n244 = Unbundle By Name(w595) -> ("TemplateClass"=w597:refnum<vi>)
            n245 = disable-structure shown="Enabled" {
              disable-tunnel: w603 -> [w612 _]
              disable-tunnel: w601 -> [w611 _]
              disable-tunnel: w596 -> [w610 _]
              disable-tunnel: w594 -> [w609 _]
              frame Disabled {
                n246 = case shown="Error" w610 {
                  selector: w610 -> [_ w617]
                  tunnel: w611 -> [_ w619]
                  tunnel: w609 -> [_ w615]
                  tunnel: w612 -> [_ w618]
                  frame No Error {
                    n247 = stacked-sequence {
                      frame #0 {
                        n248 = Wait (ms)(milliseconds to wait=u32 2) -> ()  [unwired: 1 out]
                      }
                    }
                  }
                  frame Error {
                    w623 = path "c:/GDS_Error.txt" ("file (use dialog)")
                    n249 = Unbundle(w617) -> ("code"=w614:i32, "source"=w616:string)  [unwired: 1 out]
                    n250 = Read from Text File(file (use dialog)=w623) -> (text=w620:string)  [unwired: 3 in, 3 out]
                    n251 = Format Into String(format string="       %s(%s)Code:%d:%s:%s\n", initial string=w620, w619, w618, w614, w615, w616) -> (resulting string=w622:string)  [unwired: 1 in, 1 out]
                    n252 = stacked-sequence {
                      tunnel: w622 -> [w626]
                      tunnel: w623 -> [w624]
                      frame #0 {
                        n253 = Delete(path (use dialog)=w624) -> (deleted path=w625:path)  [unwired: 4 in, 2 out]
                        n254 = Write to Text File(file (use dialog)=w625, text=w626) -> ()  [unwired: 2 in, 3 out]
                      }
                    }
                    n255 = call <vilib>:"Beep.vi"() -> ()  [unwired: 12 in]
                  }
                }
              }
              frame Enabled {
              }
            }
            n256 = Close Reference(reference=w597) -> (error out=w598:errorcluster)  [unwired: 1 in]
            n257 = case shown="No Error" w605 {
              tunnel: w595 -> [w633 _]
              tunnel: w596 -> [w631 w634]
              tunnel: [w630 w634] -> w600
              tunnel: w598 -> [_ _]
              frame No Error {
                n258 = Unbundle By Name(w633) -> ("TemplateRef"=w632:refnum<vi>)
                n259 = Close Reference(reference=w632, error in (no error)=w631) -> (error out=w630:errorcluster)
              }
              frame Error {
              }
            }
            n260 = stacked-sequence {
              tunnel: w595 -> [w629]
              tunnel: w600 -> [w627]
              tunnel: [w627] -> w599
              frame #0 {
                n261 = Unbundle By Name(w629) -> ("Class"=w628:refnum<vi>)
                n262 = call "GDSLvClass_SaveEverythingInClass.vi"("ClassRefIn"=w628) -> ()  [unwired: 17 in, 2 out]
              }
            }
          }
        }
        n263 = Equal?(x=w28, y="Exit") -> (x = y?=w31:bool)
        n264 = Select(t="Error", s=w20, f=w28) -> (s? t:f=w32:string)
      }
    }
    frame Error {
    }
  }
  "error out" <- w10
  n265 = Unbundle By Name(w6) -> ("permissions"=w2:i16, "TemplateFile"=w4:path, "TemplateVersionUsed"=→"TemplateVersionUsed":string)
  n266 = Empty String/Path?(string/path=w4) -> (empty?=w5:bool)
  n267 = case shown="False" w5 {
    tunnel: w4 -> [w637 _]
    tunnel: w2 -> [w636 _]
    frame False {
      n268 = Set Permissions(7:w636, 11:w637) -> ()  [unwired: 3 in, 2 out]
    }
    frame True {
    }
  }
